vi "Fine Frequency Synchronization.vi"(10 "Frame after fine time sync":cdb[](array[numeric]), 11 "Ts":dbl) -> (2 "Fine freq est":dbl, 3 "Frame after fine freq sync":cdb[](array[numeric]))   [LabVIEW 2024]
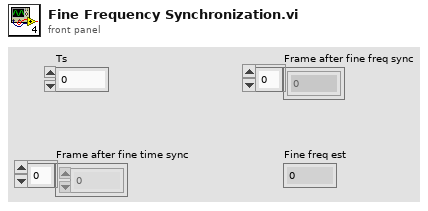
[diagram p1: front panel]
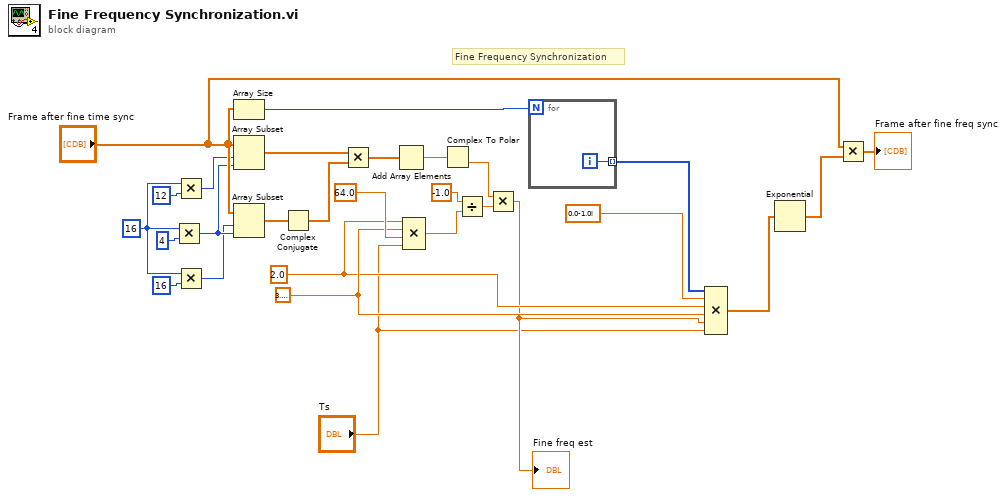
[diagram p0: block diagram]
diagram:
  w5 = 3.141592653589793
  w4 = 2.0 ("x")
  w14 = 16 ("index")
  # "Fine Frequency Synchronization"
  n1 = Multiply(x=w14, y=4) -> (x*y=w16:i32)
  n2 = Multiply(x=w14, y=12) -> (x*y=w12:i32)
  n3 = Multiply(x=w14, y=16) -> (x*y=w13:i32)
  n4 = Array Size(array="Frame after fine time sync") -> (size(s)=w28:i32)
  n5 = Array Subset(array="Frame after fine time sync", index=w12, length=w16) -> (w25:cdb[])
  n6 = Array Subset(array="Frame after fine time sync", index=w13, length=w16) -> (w17:cdb[])
  n7 = Complex Conjugate(1:w17) -> (0:w24:cdb[])
  n8 = Multiply(x=w25, y=w24) -> (x*y=w26:cdb[])
  n9 = Add Array Elements(numeric array=w26) -> (sum=w27:cdb)
  n10 = Compound Arithmetic op=MULTIPLY(w4, w5, 64.0 ("x"), "Ts") -> (w7:dbl)
  n11 = Complex To Polar(r * e^(i*theta)=w27) -> (theta=w20:dbl)  [unwired: 1 out]
  n12 = Divide(x=-1.0, y=w7) -> (x/y=w19:dbl)
  n13 = Multiply ("Multiply.vi")(x=w20, y=w19) -> (x*y=w3:dbl)
  "Fine freq est" <- w3
  n14 = for {
    N: w28 -> [_]
    tunnel: [w29] -> w9 mode=indexing
    i -> [w29]
  }
  n15 = Compound Arithmetic op=MULTIPLY(w9, cdb 0.0-1.0i ("Real Matrix A"), w4, w5, w3, "Ts") -> (w1:cdb[])
  n16 = Exponential ("Exponential.vi")(1:w1) -> (0:w21:cdb[])
  n17 = Multiply(x="Frame after fine time sync", y=w21) -> (x*y=→"Frame after fine freq sync":cdb[])
